vi "Main.vi"() -> ()   [LabVIEW 2026]
uses:
  Controls/StateType.ctl
  Controls/DataType.ctl
  Controls/ModeType.ctl
  Controls/CommandType.ctl
panel:
  out "Laps":dbl[](array[numeric])
  out "State":T1
  out "Milliseconds":dbl
  out "Seconds":dbl
  out "Minutes":dbl
  out "Hours":dbl
  in  "Quit":bool
  in  "Lap":bool
  in  "Reset":bool
  in  "Stop":bool
  in  "Start":bool
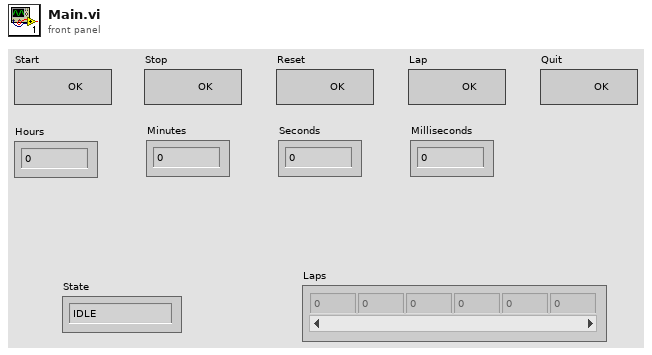
[diagram p1: front panel]
types:
  T1 = typedef "StateType.ctl" = enum16{"IDLE", "RUNNING", "PAUSED", "FINISHED"}
  T2 = typedef "DataType.ctl" = cluster{"State":T1, "RunningMode":T3, "StartTime":dbl, "AccumulatedTime":dbl, "CntDownTime":dbl, "Laps":dbl[]}
  T3 = typedef "ModeType.ctl" = enum16{"CHRONO", "COUNTDOWN", ""}
  T4 = typedef "CommandType.ctl" = enum16{"START", "STOP", "RESET", "LAP", "MODE", "TICK"}
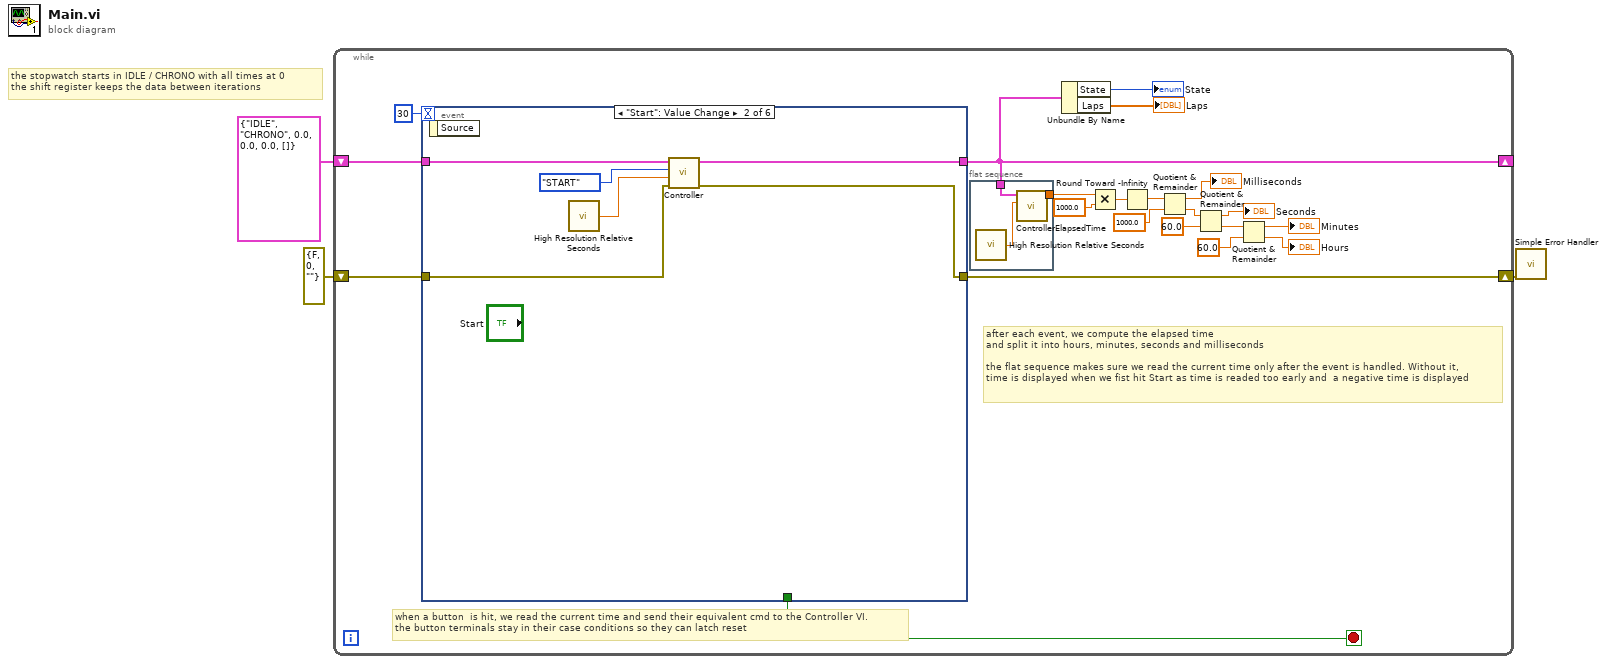
[diagram p0: block diagram]
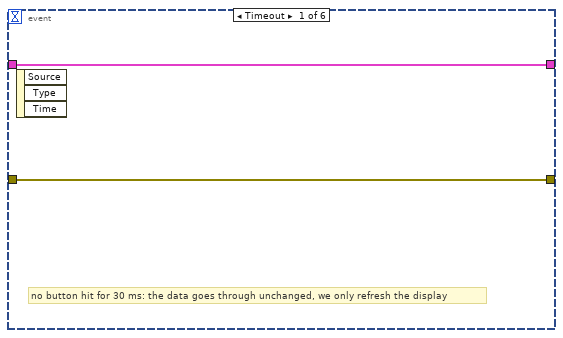
[diagram p2: hidden frame]
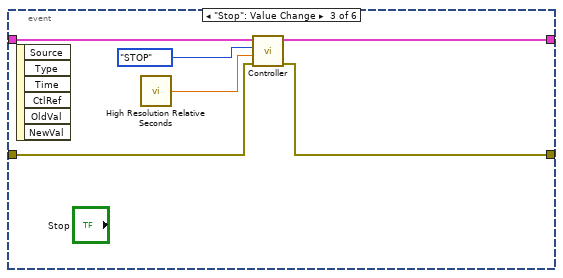
[diagram p3: hidden frame]
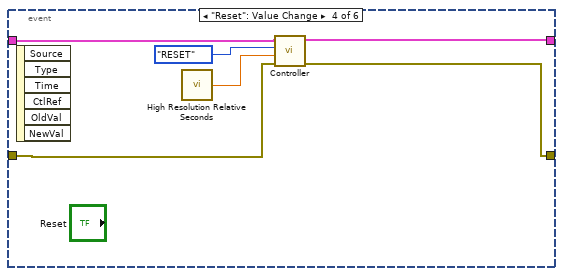
[diagram p4: hidden frame]
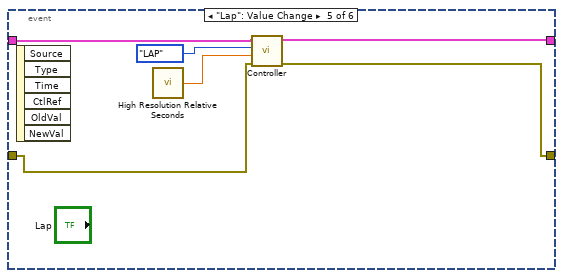
[diagram p5: hidden frame]
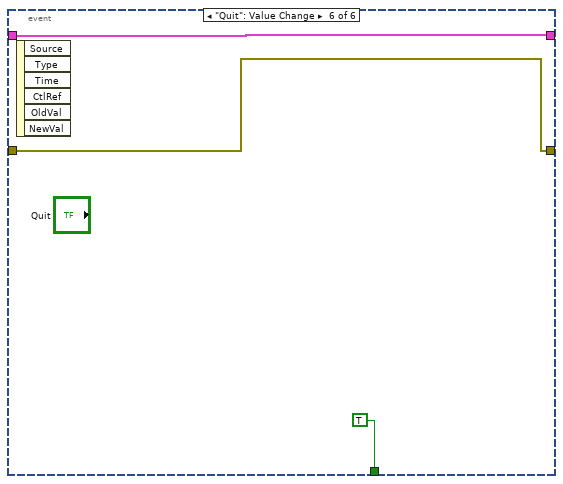
[diagram p6: hidden frame]
diagram:
  # "the stopwatch starts in IDLE / CHRONO with all times at 0\nthe shift register keeps the data between iterations"
  n1 = while {
    shift-right: [w7] -> _
    shift-left: T2 {"State"=enum."IDLE", "RunningMode"=enum."CHRONO", "StartTime"=0.0, "AccumulatedTime"=0.0, "CntDownTime"=0.0, "Laps"=[]} ("DataStructure") -> [w23]
    shift-right: [w22] -> w1
    shift-left: errorcluster {"status"=FALSE, "code"=0, "source"=""} ("error out") -> [w21]
    stop <- w4 stop-if-true
    # "after each event, we compute the elapsed time\nand split it into hours, minutes, seconds and milliseconds\n\nthe flat sequence makes sure we read the current time only after the event is handled. Without it, \ntime is displayed when we fist hit Start as time is readed too early and  a negative time is displayed"
    # "when a button  is hit, we read the current time and send their equivalent cmd to the Controller VI.\nthe button terminals stay in their case conditions so they can latch reset"
    n2 = event shown="[1] \"Start\": Value Change" {
      selector: _ -> [_ _ _ _ _ _]
      dyn-events: _ -> [_ _ _ _ _ _]
      timeout: 30 -> [_ _ _ _ _ _]
      tunnel: [w29 w30 w39 w45 w51 w55] -> w7
      tunnel: w23 -> [w29 w34 w40 w46 w52 w55]
      tunnel: [w28 w31 w38 w42 w48 w54] -> w22
      tunnel: w21 -> [w28 w32 w36 w43 w49 w54]
      tunnel: [_ _ _ _ _ TRUE] -> w4
      event Timeout {
        # "no button hit for 30 ms: the data goes through unchanged, we only refresh the display"
        n3 = event-data() -> ()  [unwired: 1 in, 3 out]
      }
      event "Start": Value Change {
        n4 = event-data() -> ()  [unwired: 1 in, 1 out]
        n5 = call <vilib>:"High Resolution Relative Seconds.vi"() -> ("relative seconds"=w33:dbl)
        n6 = call "Controller.vi"("error in"=w32, "TimeNow"=w33, "Command"=CommandType."START", "InData"=w34) -> ("error out"=w31:errorcluster, "OutData"=w30:T2)  [unwired: 6 in]
      }
      event "Stop": Value Change {
        n7 = event-data() -> ()  [unwired: 1 in, 6 out]
        n8 = call <vilib>:"High Resolution Relative Seconds.vi"() -> ("relative seconds"=w37:dbl)
        n9 = call "Controller.vi"("error in"=w36, "TimeNow"=w37, "Command"=CommandType."STOP", "InData"=w40) -> ("error out"=w38:errorcluster, "OutData"=w39:T2)  [unwired: 6 in]
      }
      event "Reset": Value Change {
        n10 = event-data() -> ()  [unwired: 1 in, 6 out]
        n11 = call <vilib>:"High Resolution Relative Seconds.vi"() -> ("relative seconds"=w44:dbl)
        n12 = call "Controller.vi"("error in"=w43, "TimeNow"=w44, "Command"=CommandType."RESET", "InData"=w46) -> ("error out"=w42:errorcluster, "OutData"=w45:T2)  [unwired: 6 in]
      }
      event "Lap": Value Change {
        n13 = event-data() -> ()  [unwired: 1 in, 6 out]
        n14 = call <vilib>:"High Resolution Relative Seconds.vi"() -> ("relative seconds"=w50:dbl)
        n15 = call "Controller.vi"("error in"=w49, "TimeNow"=w50, "Command"=CommandType."LAP", "InData"=w52) -> ("error out"=w48:errorcluster, "OutData"=w51:T2)  [unwired: 6 in]
      }
      event "Quit": Value Change {
        n16 = event-data() -> ()  [unwired: 1 in, 6 out]
      }
    }
    n17 = flat-sequence {
      tunnel: [w26] -> w20
      tunnel: w7 -> [w25]
      frame #0 {
        n18 = call <vilib>:"High Resolution Relative Seconds.vi"() -> ("relative seconds"=w27:dbl)
        n19 = call "ControllerElapsedTime.vi"("TimeNow"=w27, "InData"=w25) -> ("Elapsed"=w26:dbl)  [unwired: 9 in]
      }
    }
    n20 = Unbundle By Name(w7) -> ("State"=→"State":T1, "Laps"=→"Laps":dbl[])
    n21 = Multiply(x=w20, y=1000.0) -> (x*y=w18:dbl)
    n22 = Round Toward -Infinity(1:w18) -> (0:w17:dbl)
    n23 = Quotient & Remainder(x=w17, y=1000.0) -> (x-y*floor(x/y)=→"Milliseconds":dbl, floor(x/y)=w14:dbl)
    n24 = Quotient & Remainder(x=w14, y=60.0) -> (x-y*floor(x/y)=→"Seconds":dbl, floor(x/y)=w11:dbl)
    n25 = Quotient & Remainder(x=w11, y=60.0) -> (x-y*floor(x/y)=→"Minutes":dbl, floor(x/y)=→"Hours":dbl)
  }
  n26 = call <vilib>:"Simple Error Handler.vi"("error in (no error)"=w1) -> ()  [unwired: 4 in, 5 out]
